vi "getSerializedData.vi"(0 "reference":refnum<class "PointNode.lvclass">, 5 "error in (no error)":errorcluster) -> (14 "reference out":refnum<class "PointNode.lvclass">, 15 "parent":refnum<class "AbstractNode.lvclass">, 16 "children":refnum<class "AbstractNode.lvclass">[](array[class]), 17 "xmlOut":string, 19 "error out":errorcluster)   [LabVIEW 2020, in "PointNode.lvclass"]
doc: "getSerializedData"
uses:
  <resource>/Framework/Providers/Open_GDS/UML/PointNode_class/PointNode.lvclass
  C:/Program Files (x86)/National Instruments/LabVIEW 2020/resource/Framework/Providers/Open_GDS/UML/AbstractNode_class/AbstractNode.lvclass
  <resource>/Framework/Providers/Open_GDS/UML/AbstractNode_class/AbstractNode.lvclass
  <resource>/Framework/Providers/Open_GDS/UML/General/Point/Point Point2D.ctl
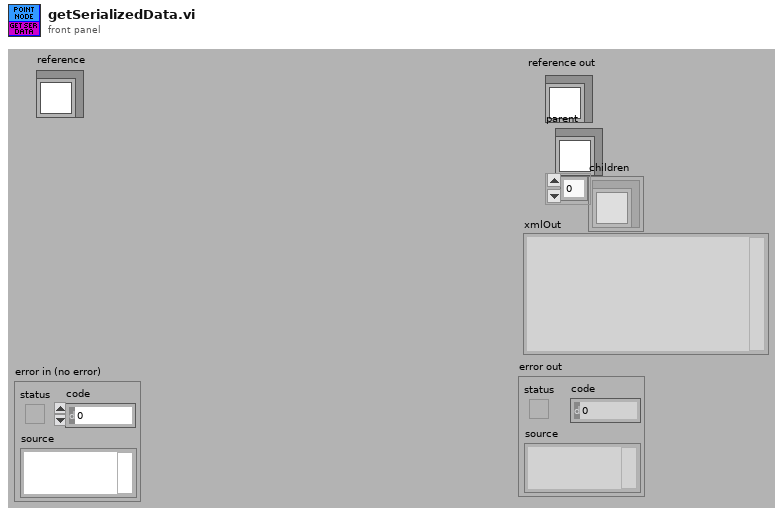
[diagram p1: front panel]
types:
  T1 = typedef "Point Point2D.ctl" = cluster{"x":dbl, "y":dbl}
  T2 = cluster{"Base class":cluster{"parent":refnum<k1>, "children":refnum<k1>[]}, "point":T1}
  T3 = typedef "PointNode.lvclass/ObjectAttributes.ctl" = cluster{"point":T1}
  T4 = typedef "AbstractNode.lvclass/ObjectAttributes.ctl" = cluster{"parent":refnum<class "AbstractNode.lvclass">, "children":refnum<class "AbstractNode.lvclass">[], "Hidden":bool}
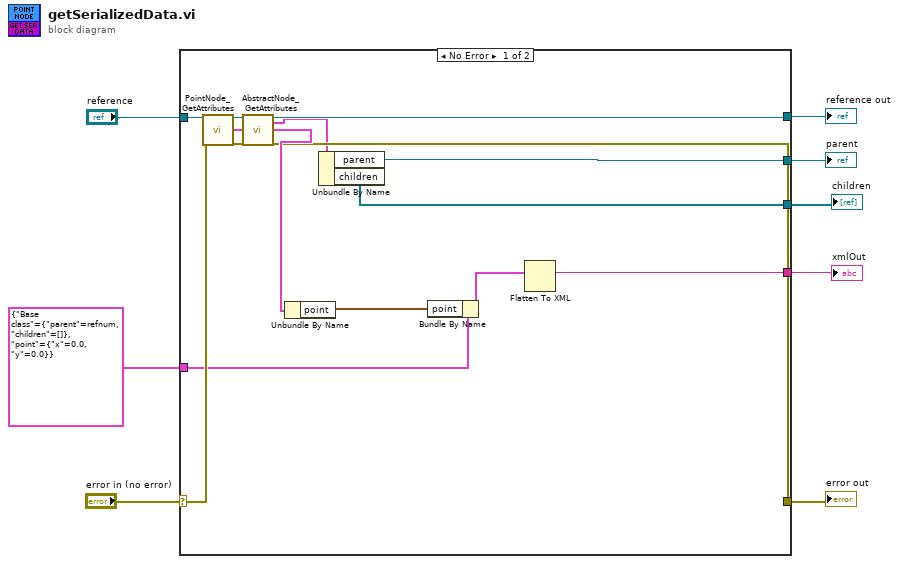
[diagram p0: block diagram]
diagram:
  n1 = case shown="No Error" "error in (no error)" {
    selector: "error in (no error)" -> [w22 w23]
    tunnel: "reference" -> [w21 w24]
    tunnel: [w11 w23] -> w6
    tunnel: [w10 w24] -> w5
    tunnel: [w20 _] -> w4
    tunnel: [w19 _] -> w3
    tunnel: [w18 _] -> w2
    tunnel: T2 {"Base class"={"parent"=refnum, "children"=[]}, "point"={"x"=0.0, "y"=0.0}} ("Attributes") -> [w17 _]
    frame No Error {
      n2 = call <resource>:"PointNode_GetAttributes.vi"("reference in"=w21, "error in (no error)"=w22) -> ("reference out"=w13:refnum<class "PointNode.lvclass">, "Data"=w14:T3, "error out"=w12:errorcluster)  [unwired: 1 in, 14 out]
      n3 = call <resource>:"AbstractNode_GetAttributes.vi"("reference in"=w13, "error in (no error)"=w12) -> ("reference out"=w10:refnum<class "PointNode.lvclass">, "Data"=w9:T4, "error out"=w11:errorcluster)  [unwired: 14 in, 1 out]
      n4 = Unbundle By Name(w14) -> ("point"=w16:T1)
      n5 = Unbundle By Name(w9) -> ("parent"=w20:refnum<class "AbstractNode.lvclass">, "children"=w19:refnum<class "AbstractNode.lvclass">[])
      n6 = Bundle By Name(cluster=w17, "point"=w16) -> (w15:T2)
      n7 = Flatten To XML(6:w15) -> (2:w18:string)
    }
    frame Error {
    }
  }
  "reference out" <- w5
  "error out" <- w6
  "parent" <- w4
  "children" <- w3
  "xmlOut" <- w2
